vi "Auto Play Path.vi"(8 "Operation":T3, 10 "(N-N-C-P) Swerve Motors":T4 {"Steer Scaling" format="%.2f"; "Drive Scaling" format="%.2f"; "Pod Locations (ft)"."Right Back Position" format="%.2f"; "Pod Locations (ft)"."Right Front Position" format="%.2f"; "Pod Locations (ft)"."Left Back Position" format="%.2f"; "Pod Locations (ft)"."Left Front Position" format="%.2f"}, 11 "Auto Data":T1) -> (0 "Auto Done?":bool, 2 "BotPose":cluster{"Numeric":dbl, "Numeric":dbl}[](array[cluster]), 3 "Bordeaux Pos":cluster{dbl, dbl}[](array[cluster]))   [LabVIEW 2023]
uses:
  Implementation/Drive Operations.ctl
  <vilib>/Rock Robotics/WPI/DriverStation/WPI_DriverStationRobotMode2.ctl
  Robot Global Data.vi
  <vilib>/REV Custom Controls/Spark Output Control Type.ctl
  <vilib>/REVLibDriver/REVLibDriver.lvlib
  <vilib>/MRC/MrcLib.lvlib
  swerve-template/Type Definitions/Data/Pod Positions.ctl
  swerve-template/Type Definitions/Data/Robot Velocities.ctl
  Implementation/Auto Data.ctl
  <vilib>/REV Custom Controls/REVSparkRefnum.ctl
  swerve-template/Type Definitions/Hardware/Swerve Drives/(NEO-NEO-ThroughBore-Pigeon2) Swerve.ctl
panel:
  out "Array":T2[](array[typedef])
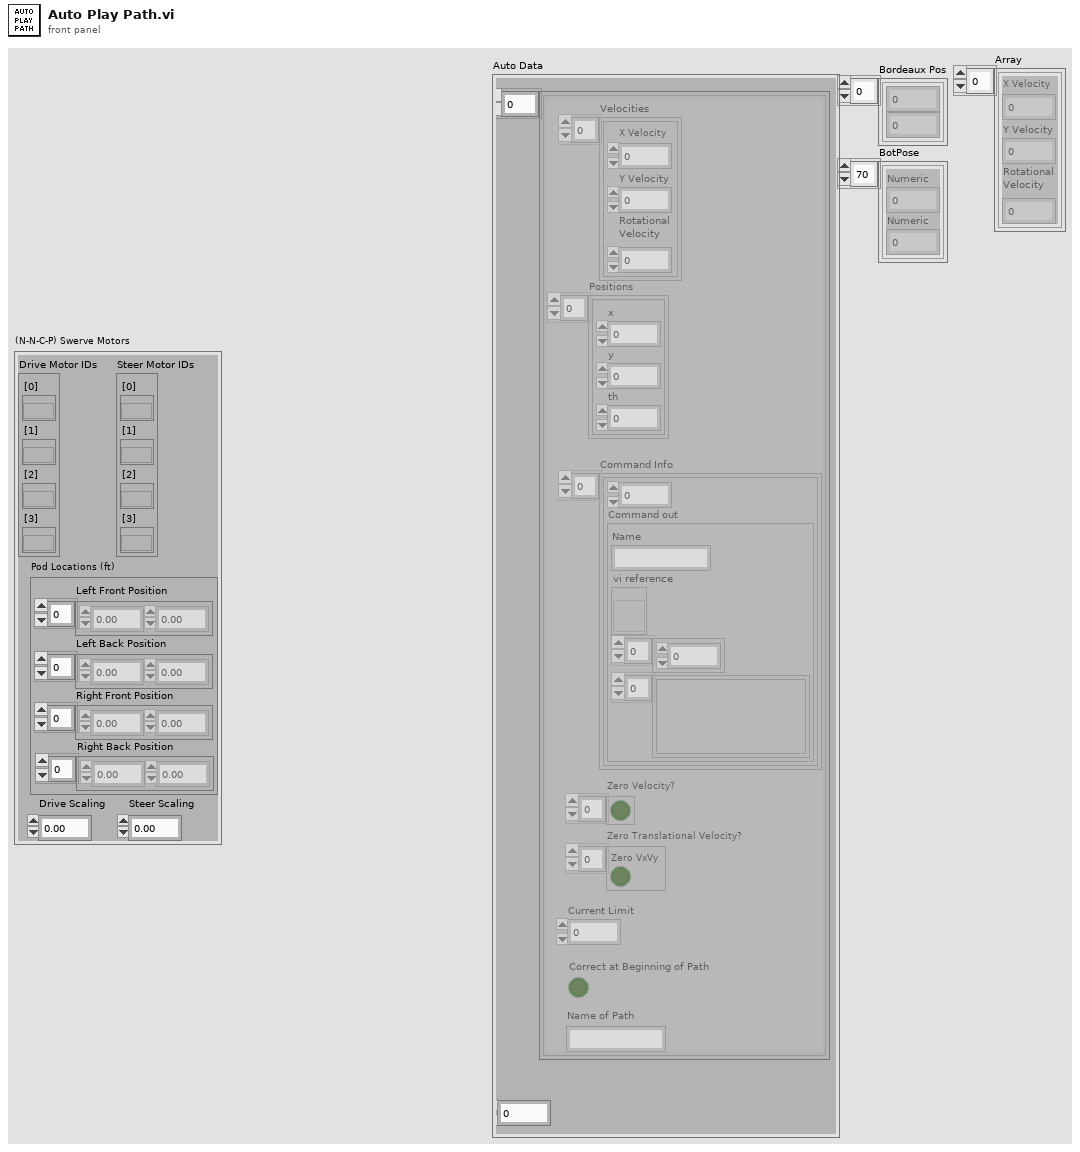
[diagram p1: front panel]
types:
  T1 = typedef "Auto Data.ctl" = cluster{"Auto Data":cluster{"Velocities":T2[], "Positions":cluster{"x":dbl, "y":dbl, "th":dbl}[], "Command Info":cluster{dbl, "Command out":cluster{"Name":string, "vi reference":refnum<vi>, i32[], variant[]}}[], "Zero Velocity?":bool[], "Zero Translational Velocity?":bool[], "Current Limit":dbl, "Correct at Beginning of Path":bool, "Name of Path":string}[], "Number of Remaining Auto Paths":dbl}
  T2 = typedef "Robot Velocities.ctl" = cluster{"X Velocity":dbl, "Y Velocity":dbl, "Rotational \nVelocity":dbl}
  T3 = typedef "Drive Operations.ctl" = enum16{"Reserve", "Read Current", "Immediate", "Calibrate", "Auto", "Auto Pickup"}
  T4 = typedef "(NEO-NEO-ThroughBore-Pigeon2) Swerve.ctl" = cluster{"Drive Motor IDs":cluster{"[0]":T5, "[1]":T5, "[2]":T5, "[3]":T5}, "Steer Motor IDs":cluster{"[0]":T5, "[1]":T5, "[2]":T5, "[3]":T5}, "Pod Locations (ft)":T6, "Drive Scaling":dbl, "Steer Scaling":dbl}
  T5 = typedef "REVLibDriver.lvlib/REVSparkRefnum.ctl" = refnum<k20>
  T6 = typedef "Pod Positions.ctl" = cluster{"Left Front Position":dbl[], "Left Back Position":dbl[], "Right Front Position":dbl[], "Right Back Position":dbl[]}
  T7 = typedef "REVLibDriver.lvlib/Spark Output Control Type.ctl" = enum16{"Percent VBus", "Velocity", "Voltage", "Position", "Current", "MAXMotion Position", "MAXMotion Velocity"}
  T8 = cluster{"Time (s)":dbl, "Command out":cluster{"Name":string, "vi reference":refnum<vi>, i32[], variant[]}}
  T9 = cluster{"Left Front":dbl, "Left Back":dbl, "Right Front":dbl, "Right Back":dbl}
  T10 = typedef "WPI_DriverStationRobotMode2.ctl" = enum16{"Autonomous Disabled", "Autonomous Enabled", "Teleop Disabled", "Teleop Enabled", "Disconnected", "Finish", "Test Disabled", "Test Enabled", "Emergency Stopped"}
  T11 = cluster{dbl, "Command out":cluster{"Name":string, "vi reference":refnum<vi>, i32[], variant[]}}[]
  T12 = typedef "Drive Conditions.ctl" = cluster{"Field Centric":bool, "Reset PIDs":bool}
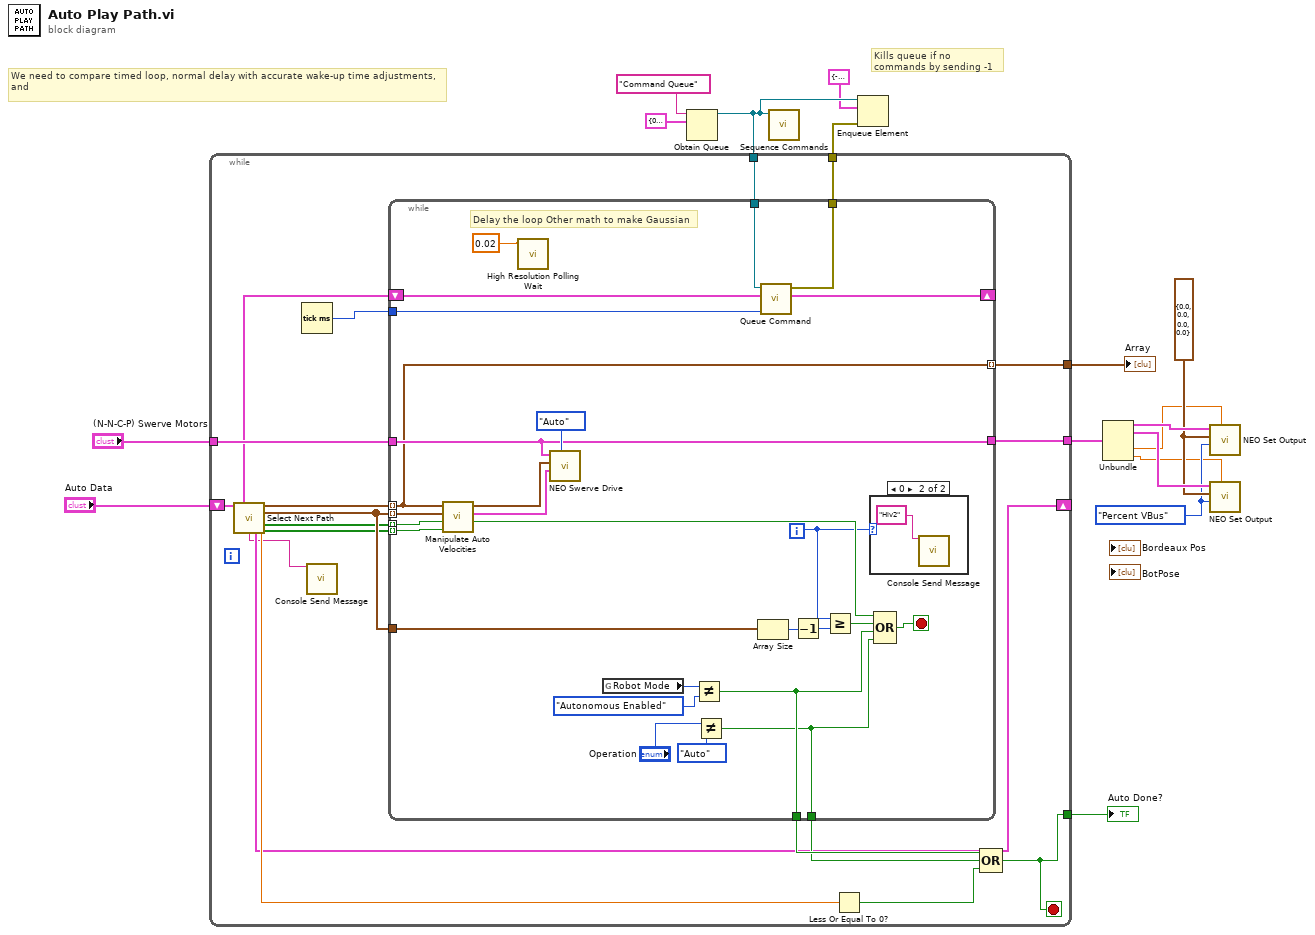
[diagram p0: block diagram]
diagram:
  w3 = Spark_Output_Control_Type."Percent VBus" ("Control Mode")
  w12 = T9 {"Left Front"=0.0, "Left Back"=0.0, "Right Front"=0.0, "Right Back"=0.0} ("Setpoints")
  # "We need to compare timed loop, normal delay with accurate wake-up time adjustments,\nand"
  # "Kills queue if no commands by sending -1"
  n1 = Obtain Queue(name (unnamed)="Command Queue", element data type=T8 {"Time (s)"=0.0, "Command out"={"Name"="", "vi reference"=refnum, [], []}} ("element")) -> (queue out=w10:refnum<queue>)  [unwired: 3 in, 2 out]
  n2 = while {
    tunnel: [w35] -> w11
    tunnel: w10 -> [w29]
    tunnel: [w28] -> w9
    tunnel: [w34] -> w7
    tunnel: [w33] -> w6
    tunnel: "(N-N-C-P) Swerve Motors" -> [w30]
    shift-right: [w19] -> _
    shift-left: "Auto Data" -> [w25]
    stop <- w33 stop-if-true
    n3 = call "Select Next Path.vi"("Auto Data"=w25) -> ("Command Info"=w23:T11, "Velocities"=w24:T2[], "Positions"=w22:cluster{"x":dbl, "y":dbl, "th":dbl}[], "Number of Remaining Auto Paths"=w20:dbl, "Zero Velocity?"=w21:bool[], "Name of Path"=w17:string, "Auto Data Out"=w19:T1, "Zero Translational Velocity?"=w18:bool[])  [unwired: 6 in, 1 out]
    n4 = Tick Count (ms)() -> (millisecond timer value=w27:u32)
    n5 = call <vilib>:"Console Send Message.vi"("Message"=w17) -> ()  [unwired: 14 in, 1 out]
    n6 = while {
      tunnel: w30 -> [w55]
      tunnel: [w55] -> w35
      tunnel: w24 -> [w54] mode=indexing
      tunnel: w22 -> [w62] mode=indexing
      tunnel: w22 -> [w61]
      tunnel: w21 -> [w59] mode=indexing
      tunnel: [w54] -> w34 mode=indexing
      tunnel: [w45] -> w32
      tunnel: [w44] -> w31
      tunnel: w27 -> [w40]
      tunnel: w29 -> [w41]
      tunnel: [w38] -> w28
      shift-right: [w39] -> _
      shift-left: w23 -> [w42]
      tunnel: w18 -> [w37] mode=indexing
      i -> [w43]
      stop <- w46 stop-if-true
      # "Delay the loop Other math to make Gaussian"
      n7 = call "Manipulate Auto Velocities.vi"("Zero Translational V"=w37, "Zero V"=w59, "Position"=w62, "Robot Velocities"=w54) -> ("Done?"=w48:bool, "Drive Conditions"=w56:T12, "Robot Velocities Out"=w53:T2)  [unwired: 5 in]
      n8 = call <vilib>:"High Resolution Polling Wait.vi"("seconds to wait"=0.02) -> ()  [unwired: 10 in, 1 out]
      n9 = call "NEO Swerve Drive.vi"("Operation"=Drive_Operations."Auto", "Drive Conditions"=w56, "Robot Velocities"=w53, "Motors In"=w55) -> ()  [unwired: 6 in, 2 out]
      n10 = global read "Robot Global Data.vi" "Robot Mode"() -> (w50:T10)
      n11 = Not Equal?(x=w50, y=WPI_DriverStationRobotMode2."Autonomous Enabled") -> (x != y?=w45:bool)
      n12 = Not Equal?(x="Operation", y=Drive_Operations."Auto") -> (x != y?=w44:bool)
      n13 = Array Size(array=w61) -> (size(s)=w57:i32)
      n14 = call "Queue Command.vi"("millisecond timer value"=w40, "Array in"=w42, "Queue in"=w41) -> ("Array out"=w39:T11, "error out"=w38:errorcluster)  [unwired: 7 in]
      n15 = Decrement(x=w57) -> (x-1=w58:i32)
      n16 = Greater Or Equal?(x=w43, y=w58) -> (x >= y?=w47:bool)
      n17 = case shown="0" w43 {
        frame Default {
        }
        frame 0 {
          n18 = call <vilib>:"Console Send Message.vi"("Message"="Hiv2") -> ()  [unwired: 14 in, 1 out]
        }
      }
      n19 = Compound Arithmetic op=OR(w48, w47, w45, w44) -> (w46:bool)
    }
    n20 = Less Or Equal To 0?(x=w20) -> (x <= 0?=w26:bool)
    n21 = Compound Arithmetic op=OR(w32, w31, w26) -> (w33:bool)
  }
  "Auto Done?" <- w6
  "Array" <- w7
  n22 = call "Sequence Commands.vi"("queue in"=w10) -> ()  [unwired: 11 in]
  n23 = Enqueue Element(queue=w10, element=T8 {"Time (s)"=-1.0, "Command out"={"Name"="", "vi reference"=refnum, [], []}}, error in (no error)=w9) -> ()  [unwired: 1 in, 3 out]
  n24 = Unbundle(w11) -> ("Drive Motor IDs"=w14:cluster{"[0]":T5, "[1]":T5, "[2]":T5, "[3]":T5}, "Steer Motor IDs"=w13:cluster{"[0]":T5, "[1]":T5, "[2]":T5, "[3]":T5}, "Drive Scaling"=w2:dbl, "Steer Scaling"=w1:dbl)  [unwired: 1 out]
  n25 = call "NEO Set Output.vi"("Scaling"=w2, "Control Mode"=w3, "Setpoints"=w12, "Motors"=w14) -> ()  [unwired: 7 in, 1 out]
  n26 = call "NEO Set Output.vi"("Scaling"=w1, "Control Mode"=w3, "Setpoints"=w12, "Motors"=w13) -> ()  [unwired: 7 in, 1 out]
